vi "Main.vi"(9 "Tree Sync Refs":refnum<vi>[](array[refnum]), 10 "Tree Ref":refnum<vi>, 11 "Module Admin":refnum<class "Delacor_lib_QMH_Cloneable Module Admin.lvclass">) -> ()   [LabVIEW 2023, in "Tree Handlr.lvlib"]
doc: "This template is based off of the Queued Message Handler design pattern and the Queued Message Handler project template that ships with LabVIEW.\n\nThe main difference is that the queue is private to this module and communication between modules is performed via Broadcast and Request events.\n\nRequest events are wrapped in public API methods and are handled in the Event Handling Loop (EHL) of this VI. Any module can register for Broadcast events sent by this module. The EHL generates messages based on user interface actions.\n\nThe Message Handling Loop (MHL) processes messages generated by the EHL, or by other messages. The messages are string values, so new messages can be added easily to the Message Cases case structure in the MHL. Each message cluster can also provide an optional value for Message Data, which is a variant that can be converted to whatever message-specific data is required.\n_____\nBased on DQMH Project Template 7.0.1.1316."
uses:
  Tree Handlr.lvlib
  <vilib>/Delacor/Delacor QMH/Libraries/Cloneable Module Admin_class/Delacor_lib_QMH_Cloneable Module Admin.lvclass
  Module Data--cluster.ctl
  <vilib>/Delacor/Delacor QMH/Libraries/Message Queue_class/Delacor_lib_QMH_Message Queue.lvclass/Delacor_lib_QMH_Message Queue.ctl
  <vilib>/Delacor/Delacor QMH/Libraries/Cloneable Module Admin_class/Delacor_lib_QMH_Cloneable Module Admin.lvclass/Delacor_lib_QMH_Cloneable Module Admin.ctl
  Stop Argument--cluster.ctl
  <vilib>/Delacor/Delacor QMH/Libraries/Module Admin_class/Delacor_lib_QMH_Module Admin.lvclass/Delacor_lib_QMH_Module Admin.ctl
  Restore Open Items Argument--cluster.ctl
  <vilib>/Utility/miscctls.llb/LVPointTypeDef.ctl
  <vilib>/Delacor/Delacor QMH/Libraries/Message Queue_class/Delacor_lib_QMH_Enqueue Message (Multiline).vi
  <vilib>/Delacor/Delacor QMH/Libraries/Cloneable Module Admin_class/Delacor_lib_QMH_Get Module ID.vi
  <vilib>/Delacor/Delacor QMH/Libraries/Module Admin_class/Delacor_lib_QMH_Get External Launch.vi
  LabVIEW-common/TEMPLATES/State Machine/State Machine Sub/Process Multi-LineState String.vi
  <vilib>/Utility/inputDevices.llb/keyboardAcquire.vi
  <vilib>/Delacor/Delacor QMH/Libraries/Message Queue_class/Delacor_lib_QMH_Message Queue.lvclass
panel:
  out "error out":errorcluster
  out "Status":string
  in  "Simulate EHL Error":bool
  in  "Simulate MHL Error":bool
  # "Other processes communicate with this Module via its Public API (wrappers for its Request Events).\n\nThis Module communicates with other processes via its Broadcast Events.\nAny process that wants to receive these messages can register for this module's Broadcast events."
  # "This template is for the DQMH framework. See the block diagram for more information on how to use this template."
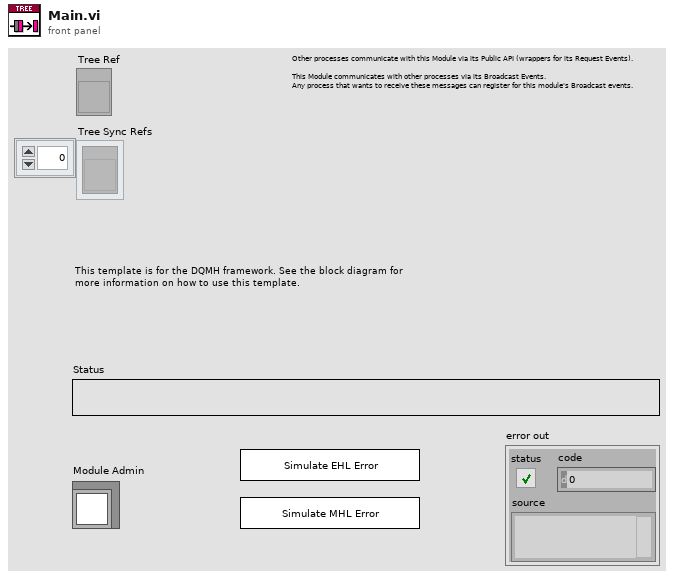
[diagram p1: front panel]
types:
  T1 = typedef "Tree Handlr.lvlib/Request Events--cluster.ctl" = cluster{"Stop Module":refnum<user-event>, "Show Panel":refnum<user-event>, "Hide Panel":refnum<user-event>, "Show Diagram":refnum<user-event>, "Get Module Execution Status":refnum<user-event>, "Restore Open Items":refnum<user-event>, "Record Open Items":refnum<user-event>}
  T2 = typedef "Tree Handlr.lvlib/Module Data--cluster.ctl" = cluster{"Status":string}
  T3 = enum32{"invalid lock state", "Not Locked", "Locked (No Password)", "Password-protected"}
  T4 = typedef "Tree Handlr.lvlib/Stop Argument--cluster.ctl" = cluster{"Module ID":i32, "Origin":string, "Exit via Stop Module Req?":bool, "Wait for Module to stop?":bool}
  T5 = enum16{"0", "1", "2", "3", "4", "5", "6", "7", "8", "9", "A", "B", "C", "D", "E", "F", "G", "H", "I", "J", "K", "L", "M", "N", "O", "P", "Q", "R", "S", "T", "U", "V", "W", "X", "Y", "Z", "F1", "F2", "F3", "F4", "F5", "F6", "F7", "F8", "F9", "F10", "F11", "F12", "F13", "F14", "F15", "ADD", "BACK", "BACKSLASH", "CAPITAL", "COMMA", "DECIMAL", "DELETE", "DIVIDE", "DOWN", "END", "EQUALS", "ESCAPE", "GRAVE (`)", "HOME", "INSERT", "LBRACKET", "LCONTROL", "LEFT", "L ALT", "LSHIFT", "LWIN", "MINUS", "MULTIPLY", "NEXT", "NUMLOCK", "NUMPAD_0", "NUMPAD_1", "NUMPAD_2", "NUMPAD_3", "NUMPAD_4", "NUMPAD_5", "NUMPAD_6", "NUMPAD_7", "NUMPAD_8", "NUMPAD_9", "PAUSE", "PERIOD", "PRIOR (PG UP)", "RBRACKET", "RCONTROL", "RETURN", "RIGHT", "R ALT", "RSHIFT", "RWIN", "SCROLL", "SEMICOLON", "SLASH", "SPACE", "SUBTRACT", "TAB", "UP", "ENTER (num pad)", "' (quote)"}
  T6 = typedef "Tree Handlr.lvlib/Restore Open Items Argument--cluster.ctl" = cluster{"Module ID":i32, "Boolean":bool}
  T7 = typedef "LVPointTypeDef.ctl" = cluster{"Horizontal":i16, "Vertical":i16}
  T8 = enum32{"Invalid", "Standard", "Closed", "Hidden", "Minimized", "Maximized"}
  T9 = enum16{"0", "1", "2", "3", "4", "5", "6", "7", "8", "9", "A", "B", "C", "D", "E", "F", "G", "H", "I", "J", "K", "L", "M", "N", "O", "P", "Q", "R", "S", "T", "U", "V", "W", "X", "Y", "Z", "F1", "F2", "F3", "F4", "F5", "F6", "F7", "F8", "F9", "F10", "F11", "F12", "F13", "F14", "F15", "ADD", "BACK", "BACKSLASH", "CAPITAL", "COMMA", "DECIMAL", "DELETE", "DIVIDE", "DOWN", "END", "EQUALS", "ESCAPE", "GRAVE (`)", "HOME", "INSERT", "LBRACKET", "LCONTROL", "LEFT", "L ALT", "LSHIFT", "LWIN", "MINUS", "MULTIPLY", "NEXT", "NUMLOCK", "NUMPAD_0", "NUMPAD_1", "NUMPAD_2", "NUMPAD_3", "NUMPAD_4", "NUMPAD_5", "NUMPAD_6", "NUMPAD_7", "NUMPAD_8", "NUMPAD_9", "PAUSE", "PERIOD", "PRIOR (PG UP)", "RBRACKET", "RCONTROL", "RETURN", "RIGHT", "R ALT", "RSHIFT", "RWIN", "SCROLL", "SEMICOLON", "SLASH", "SPACE", "SUBTRACT", "TAB", "UP", "ENTER (num pad)", "' (quote)"}[]
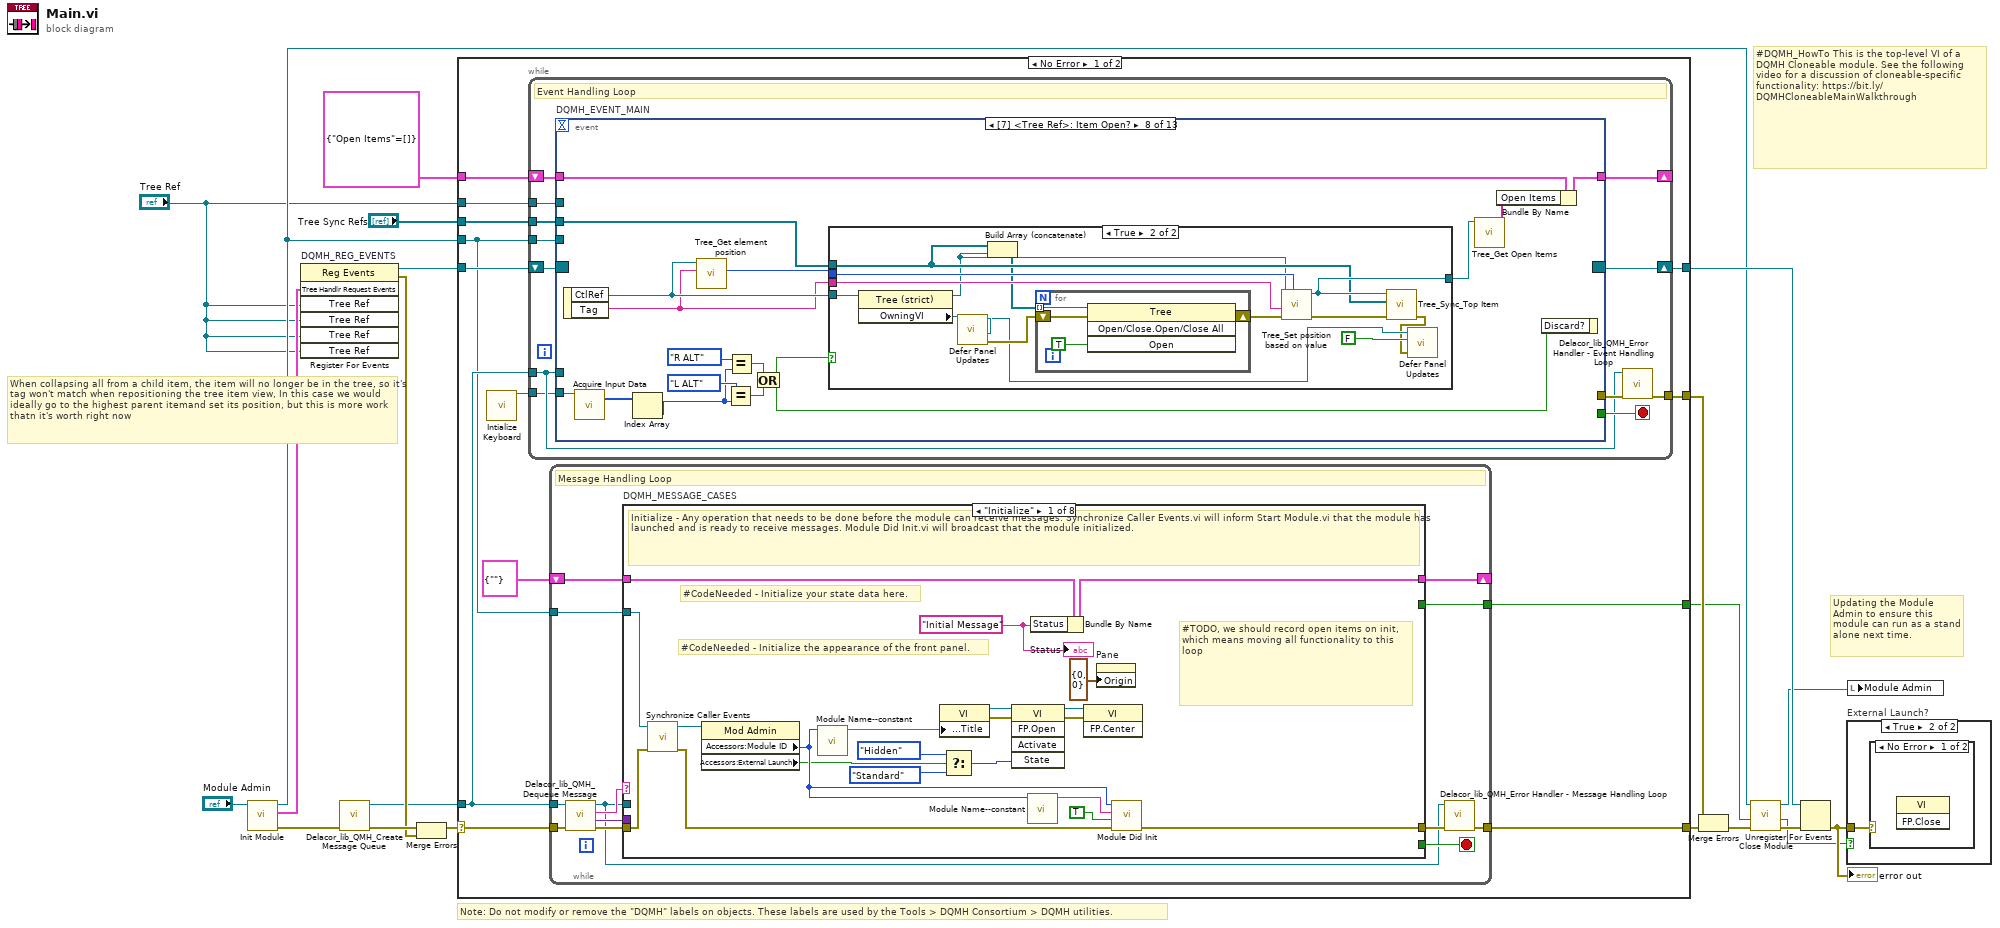
[diagram p0: block diagram]
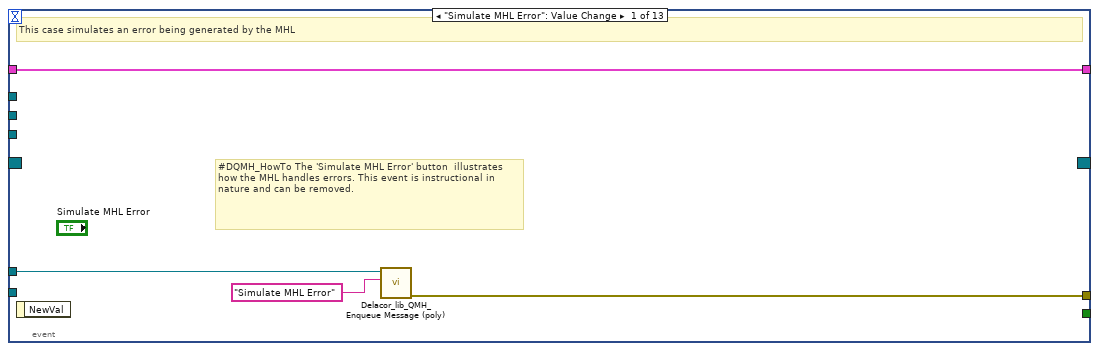
[diagram p2: hidden frame]
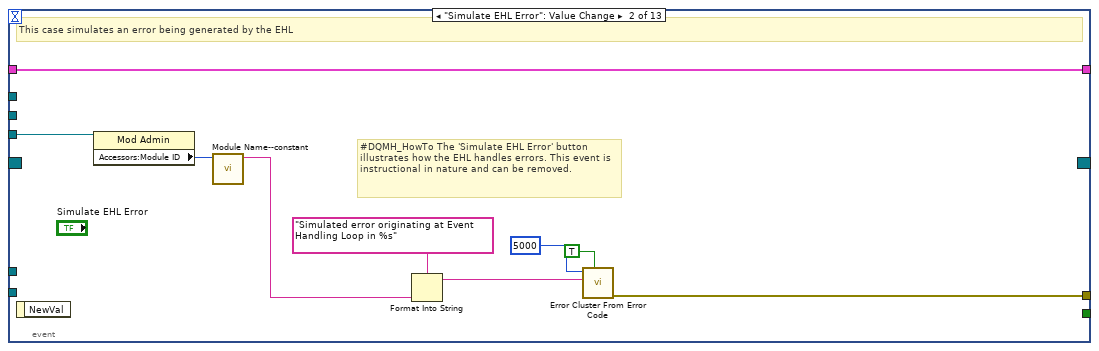
[diagram p3: hidden frame]
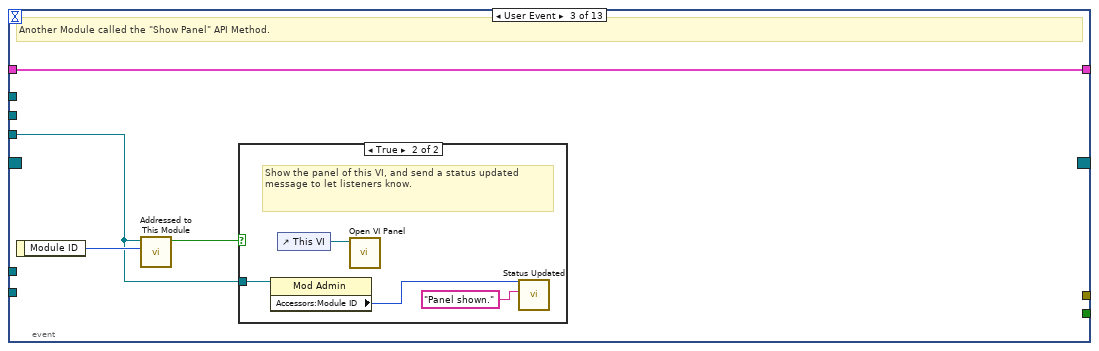
[diagram p4: hidden frame]
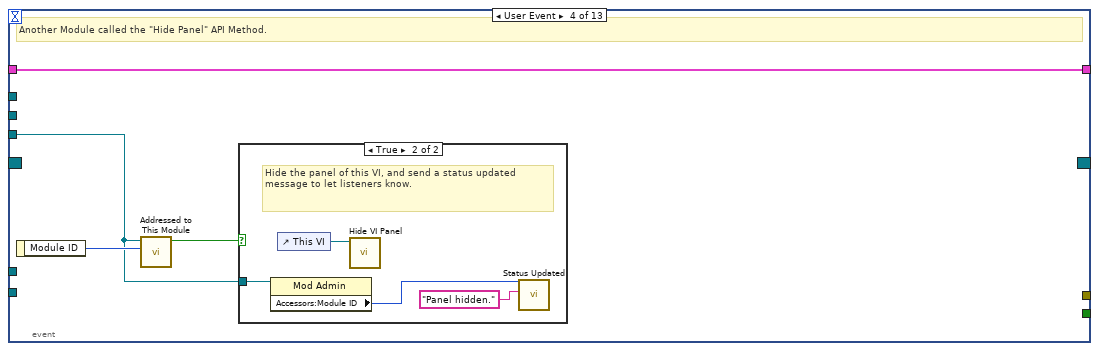
[diagram p6: hidden frame]
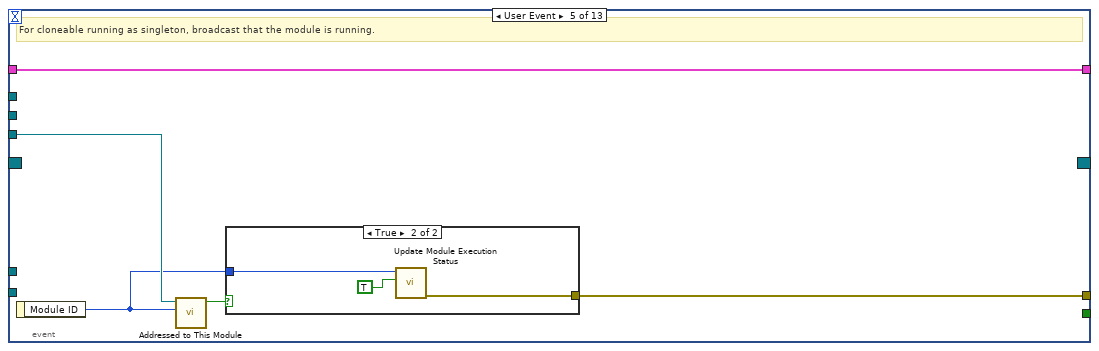
[diagram p8: hidden frame]
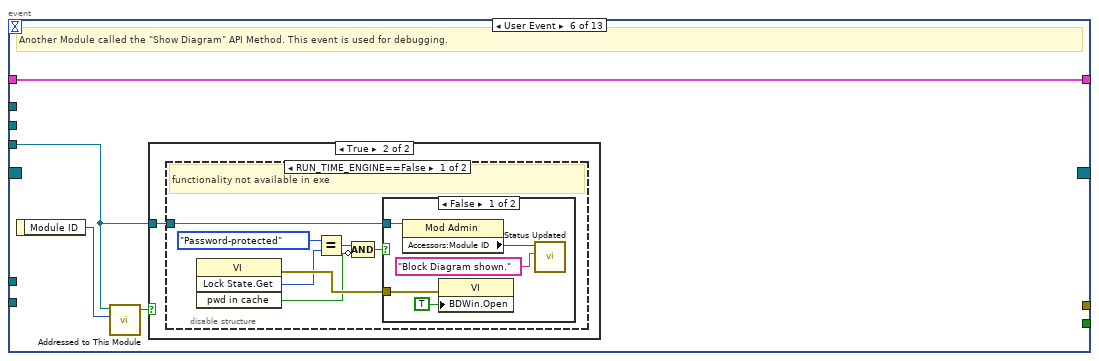
[diagram p10: hidden frame]
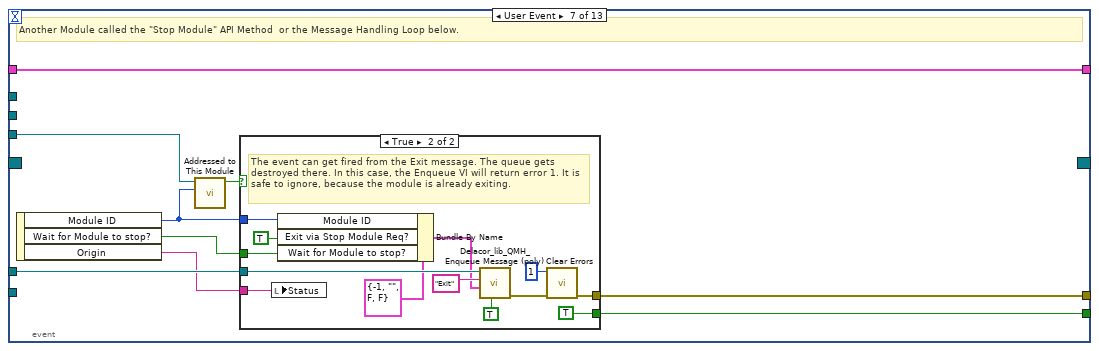
[diagram p14: hidden frame]
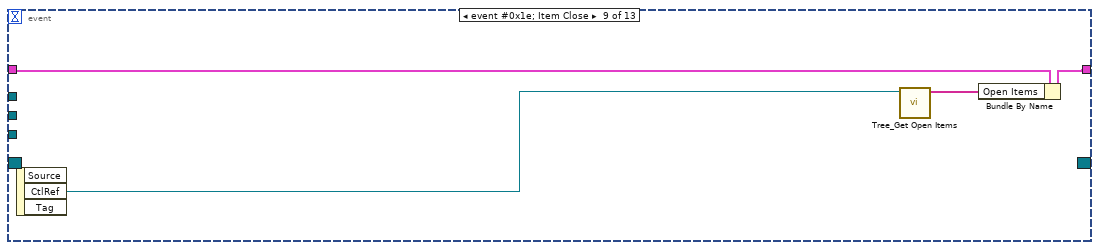
[diagram p17: hidden frame]
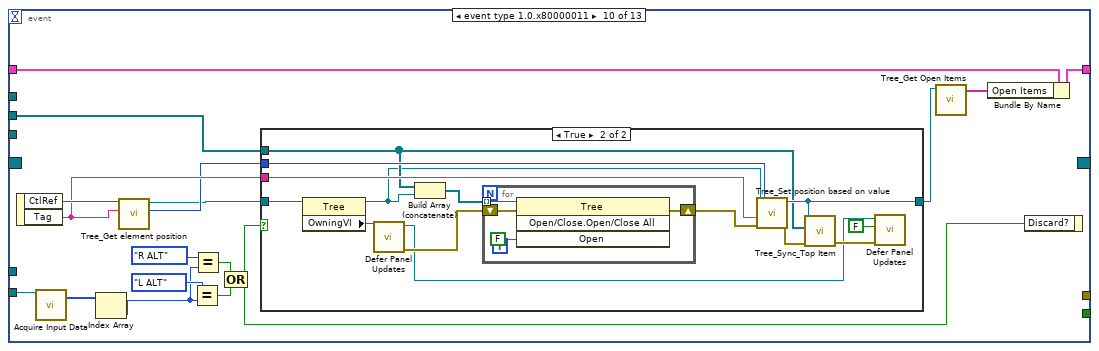
[diagram p18: hidden frame]
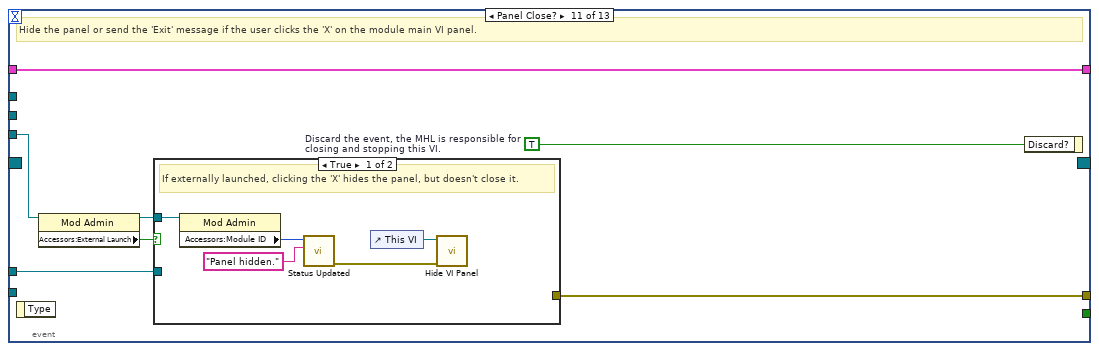
[diagram p20: hidden frame]
diagram:
  # "When collapsing all from a child item, the item will no longer be in the tree, so it's tag won't match when repositioning the tree item view, In this case we would ideally go to the highest parent itemand set its position, but this is more work thatn it's worth right now"
  # "#DQMH_HowTo This is the top-level VI of a DQMH Cloneable module. See the following video for a discussion of cloneable-specific functionality: https://bit.ly/DQMHCloneableMainWalkthrough"
  # "Note: Do not modify or remove the \"DQMH\" labels on objects. These labels are used by the Tools > DQMH Consortium > DQMH utilities."
  # "Updating the Module Admin to ensure this module can run as a stand alone next time."
  n1 = call "Init Module.vi"("Cloneable Module Admin in"="Module Admin") -> ("error out"=w18:errorcluster, "Tree Handlr Request Events"=w10:T1, "Cloneable Module Admin out"=w7:refnum<class "Delacor_lib_QMH_Cloneable Module Admin.lvclass">)  [unwired: 8 in]
  n2 = register-events "DQMH_REG_EVENTS"(w10, "Tree Ref", "Tree Ref", "Tree Ref", "Tree Ref") -> (reference out=w11:refnum<event-registration>, error out=w13:errorcluster)  [unwired: 2 in]
  n3 = call <vilib>:"Delacor_lib_QMH_Create Message Queue.vi"("error in"=w18) -> ("error out"=w15:errorcluster, "Message Queue"=w9:refnum<class "Delacor_lib_QMH_Message Queue.lvclass">)  [unwired: 9 in]
  n4 = Merge Errors(w15, w13) -> (w14:errorcluster)
  n5 = case shown="No Error" w14 {
    selector: w14 -> [w32 w347]
    tunnel: [w34 w346] -> w19
    tunnel: [w31 w345] -> w12
    tunnel: w11 -> [w29 w345]
    tunnel: w9 -> [w28 w338]
    tunnel: [w33 _] -> w20
    tunnel: w7 -> [w27 w341]
    tunnel: [w26 _] -> w5
    tunnel: cluster{"Open Items":string[]} {"Open Items"=[]} -> [w24 _]
    tunnel: "Tree Ref" -> [w23 _]
    tunnel: "Tree Sync Refs" -> [w22 _]
    frame No Error {
      n6 = call <vilib>:"Intialize Keyboard.vi"() -> ("device ID"=w25:refnum<k1>)  [unwired: 10 in, 1 out]
      n7 = while {
        tunnel: w28 -> [w40]
        shift-right: [w43] -> w31
        shift-left: w29 -> [w44]
        tunnel: [w45] -> w33
        tunnel: w27 -> [w41]
        tunnel: w25 -> [w39]
        shift-right: [w37] -> _
        shift-left: w24 -> [w38]
        tunnel: w23 -> [w36]
        tunnel: w22 -> [w35]
        stop <- w42 stop-if-true
        # "Event Handling Loop"
        n8 = event "DQMH_EVENT_MAIN" shown="[7] <Tree Ref>: Item Open?" {
          selector: w44 -> [_ _ _ _ _ _ _ _ _ _ _ _ _]
          dyn-events: [_ _ _ _ _ _ _ _ _ _ _ _ _] -> w43
          timeout: _ -> [_ _ _ _ _ _ _ _ _ _ _ _ _]
          tunnel: [_ _ _ _ _ _ w105 _ _ _ _ _ _] -> w42
          tunnel: w40 -> [w49 _ _ _ _ _ w108 _ _ _ w201 w223 _]
          tunnel: [w50 w59 _ _ w80 _ w109 _ _ _ w204 _ _] -> w46
          tunnel: w41 -> [_ w58 w61 w69 w78 w85 w107 _ _ _ w202 w221 w233]
          tunnel: w39 -> [_ _ _ _ _ _ _ w132 _ w172 _ _ _]
          tunnel: w38 -> [w47 w51 w60 w68 w76 w84 w101 w127 w161 w167 w198 w215 w231]
          tunnel: [w47 w51 w60 w68 w76 w84 w101 w126 w160 w166 w198 w214 w230] -> w37
          tunnel: w36 -> [_ _ _ _ _ _ _ _ _ _ _ w216 w229]
          tunnel: w35 -> [_ _ _ _ _ _ _ w123 _ w162 _ _ _]
          event "Simulate MHL Error": Value Change {
            # "#DQMH_HowTo The 'Simulate MHL Error' button  illustrates how the MHL handles errors. This event is instructional in nature and can be removed."
            # "This case simulates an error being generated by the MHL"
            n9 = event-data() -> ()  [unwired: 1 in, 1 out]
            n10 = call-poly <vilib>:"Delacor_lib_QMH_Enqueue Message (poly).vi"("Message"="Simulate MHL Error", "Message Queue in"=w49) -> ("error out"=w50:errorcluster)  [unwired: 8 in, 1 out]
          }
          event "Simulate EHL Error": Value Change {
            # "#DQMH_HowTo The 'Simulate EHL Error' button  illustrates how the EHL handles errors. This event is instructional in nature and can be removed."
            # "This case simulates an error being generated by the EHL"
            n11 = event-data() -> ()  [unwired: 1 in, 1 out]
            n12 = property on="Property Node" class="Mod Admin"(reference=w58) -> ("Accessors:Module ID"=w57:i32)  [unwired: 1 in, 2 out]
            n13 = call "Module Name--constant.vi"("Module ID"=w57) -> ("Module Name"=w52:string)  [unwired: 10 in]
            n14 = Format Into String(format string="Simulated error originating at Event Handling Loop in %s", w52) -> (resulting string=w55:string)  [unwired: 2 in, 1 out]
            n15 = call <vilib>:"Error Cluster From Error Code.vi"("show call chain? (False)"=TRUE, "error message (\"\")"=w55, "error code (0)"=5000) -> ("error out"=w59:errorcluster)  [unwired: 6 in]
          }
          event User Event {
            # "Another Module called the \"Show Panel\" API Method."
            n16 = event-data() -> ("Module ID"=w62:i32)  [unwired: 1 in]
            n17 = call "Addressed to This Module.vi"("Module ID from Argument"=w62, "Module Admin"=w61) -> ("Addressed to this instance?"=w63:bool)  [unwired: 8 in, 1 out]
            n18 = case shown="True" w63 {
              tunnel: w61 -> [_ w65]
              frame False {
              }
              frame True {
                # "Show the panel of this VI, and send a status updated message to let listeners know."
                n19 = property on="Property Node" class="Mod Admin"(reference=w65) -> ("Accessors:Module ID"=w64:i32)  [unwired: 1 in, 2 out]
                n20 = control-ref of="This VI"() -> (w67:refnum<vi>)
                n21 = call "Open VI Panel.vi"("VI"=w67) -> ()  [unwired: 10 in, 1 out]
                n22 = call "Status Updated.vi"("Status"="Panel shown." ("format string"), "Module ID"=w64) -> ()  [unwired: 9 in, 1 out]
              }
            }
          }
          event User Event {
            # "Another Module called the \"Hide Panel\" API Method."
            n23 = event-data() -> ("Module ID"=w70:i32)  [unwired: 1 in]
            n24 = call "Addressed to This Module.vi"("Module ID from Argument"=w70, "Module Admin"=w69) -> ("Addressed to this instance?"=w71:bool)  [unwired: 8 in, 1 out]
            n25 = case shown="True" w71 {
              tunnel: w69 -> [_ w73]
              frame False {
              }
              frame True {
                # "Hide the panel of this VI, and send a status updated message to let listeners know."
                n26 = property on="Property Node" class="Mod Admin"(reference=w73) -> ("Accessors:Module ID"=w72:i32)  [unwired: 1 in, 2 out]
                n27 = control-ref of="This VI"() -> (w75:refnum<vi>)
                n28 = call "Hide VI Panel.vi"("VI"=w75) -> ()  [unwired: 10 in, 1 out]
                n29 = call "Status Updated.vi"("Status"="Panel hidden." ("format string"), "Module ID"=w72) -> ()  [unwired: 9 in, 1 out]
              }
            }
          }
          event User Event {
            # "For cloneable running as singleton, broadcast that the module is running."
            n30 = event-data() -> ("Module ID"=w77:i32)  [unwired: 1 in]
            n31 = call "Addressed to This Module.vi"("Module ID from Argument"=w77, "Module Admin"=w78) -> ("Addressed to this instance?"=w79:bool)  [unwired: 8 in, 1 out]
            n32 = case shown="True" w79 {
              tunnel: [_ w83] -> w80
              tunnel: w77 -> [_ w82]
              frame False {
              }
              frame True {
                n33 = call "Update Module Execution Status.vi"("Running?"=TRUE, "Module ID"=w82) -> ("error out"=w83:errorcluster)  [unwired: 9 in]
              }
            }
          }
          event User Event {
            # "Another Module called the \"Show Diagram\" API Method. This event is used for debugging."
            n34 = event-data() -> ("Module ID"=w86:i32)  [unwired: 1 in]
            n35 = call "Addressed to This Module.vi"("Module ID from Argument"=w86, "Module Admin"=w85) -> ("Addressed to this instance?"=w87:bool)  [unwired: 8 in, 1 out]
            n36 = case shown="True" w87 {
              tunnel: w85 -> [_ w88]
              frame False {
              }
              frame True {
                n37 = disable-structure shown="RUN_TIME_ENGINE==False" {
                  disable-tunnel: w88 -> [w89 _]
                  frame condition #0 (active) {
                    # "functionality not available in exe"
                    n38 = invoke on="Invoke Node" class="VI" method="Lock State.Get"() -> (error out=w95:errorcluster, "Get Lock State"=w94:T3, "pwd in cache"=w91:bool)  [unwired: 4 in, 1 out]
                    n39 = Equal?(x=T3."Password-protected", y=w94) -> (x = y?=w92:bool)
                    n40 = Compound Arithmetic op=AND(w92, invert w91) -> (w90:bool)
                    n41 = case shown="False" w90 {
                      tunnel: w95 -> [w100 _]
                      tunnel: w89 -> [w97 _]
                      frame False {
                        n42 = property on="Property Node" class="Mod Admin"(reference=w97) -> ("Accessors:Module ID"=w96:i32)  [unwired: 1 in, 2 out]
                        n43 = property on="Property Node" class="VI"(error in=w100, "BDWin.Open"=TRUE ("Block Diagram Window:Open")) -> ()  [unwired: 1 in, 2 out]
                        n44 = call "Status Updated.vi"("Status"="Block Diagram shown." ("format string"), "Module ID"=w96) -> ()  [unwired: 9 in, 1 out]
                      }
                      frame True {
                        # "Password-protected VI, and the password is not in the cache. Do not show the diagram."
                      }
                    }
                  }
                  frame condition #1 {
                  }
                }
              }
            }
          }
          event User Event {
            # "Another Module called the \"Stop Module\" API Method  or the Message Handling Loop below."
            n45 = event-data() -> ("Module ID"=w103:i32, "Wait for Module to stop?"=w104:bool, "Origin"=w102:string)  [unwired: 1 in]
            n46 = call "Addressed to This Module.vi"("Module ID from Argument"=w103, "Module Admin"=w107) -> ("Addressed to this instance?"=w106:bool)  [unwired: 8 in, 1 out]
            n47 = case shown="True" w106 {
              tunnel: [_ w121] -> w109
              tunnel: w108 -> [_ w117]
              tunnel: [_ TRUE] -> w105
              tunnel: w104 -> [_ w112]
              tunnel: w103 -> [_ w114]
              tunnel: w102 -> [_ w110]
              frame False {
              }
              frame True {
                # "The event can get fired from the Exit message. The queue gets destroyed there. In this case, the Enqueue VI will return error 1. It is safe to ignore, because the module is already exiting."
                n48 = local write "Status"(w110) -> ()
                n49 = Bundle By Name(cluster=T4 {"Module ID"=-1, "Origin"="", "Exit via Stop Module Req?"=FALSE, "Wait for Module to stop?"=FALSE} ("Stop Argument"), "Module ID"=w114, "Exit via Stop Module Req?"=TRUE, "Wait for Module to stop?"=w112) -> (w111:T4)
                n50 = call-poly <vilib>:"Delacor_lib_QMH_Enqueue Message (poly).vi"("Priority Message? (F)"=TRUE, "Message Data"=w111, "Message"="Exit", "Message Queue in"=w117) -> ("error out"=w122:errorcluster)  [unwired: 6 in, 1 out]
                n51 = call <vilib>:"Clear Errors.vi"("error in (no error)"=w122, "specific error code to clear (0: all)"=1) -> ("error out"=w121:errorcluster)  [unwired: 4 in, 1 out]
              }
            }
          }
          event Item Open? {
            n52 = event-data() -> ("CtlRef"=w130:refnum<vi>, "Tag"=w129:string)  [unwired: 1 in]
            n53 = call-poly <vilib>:"Acquire Input Data.vi"("device ID"=w132) -> ("keys pressed"=w138:T9)  [unwired: 16 in, 2 out]
            n54 = Index Array(array=w138) -> (element=w135:T5)  [unwired: 1 in]
            n55 = call "Tree_Get element position.vi"("tag"=w129, "Tree Ref In"=w130) -> ("Tree Item Row"=w128:i32)  [unwired: 7 in, 2 out]
            n56 = Equal?(x=T5."L ALT" ("element"), y=w135) -> (x = y?=w133:bool)
            n57 = Equal?(x=T5."R ALT" ("element"), y=w135) -> (x = y?=w134:bool)
            n58 = Compound Arithmetic op=OR(w134, w133) -> (w131:bool)
            n59 = case shown="True" w131 {
              tunnel: w129 -> [_ w153]
              tunnel: w130 -> [w139 w149]
              tunnel: w128 -> [_ w146]
              tunnel: [w139 w143] -> w124
              tunnel: w123 -> [_ w142]
              frame False {
              }
              frame True {
                n60 = property class="Tree (strict)"(reference=w149) -> (reference out=w140:refnum<vi>, "OwningVI"=w148:refnum<vi>)  [unwired: 1 in, 1 out]
                n61 = call "Defer Panel Updates.vi"("VI Ref"=w148) -> ("error out"=w151:errorcluster, "VI Ref Out"=w147:refnum<vi>)  [unwired: 9 in]
                n62 = Build Array (concatenate)(w142, w140) -> (w141:refnum<vi>[])
                n63 = for {
                  shift-right: [w155] -> w150
                  shift-left: w151 -> [w156]
                  tunnel: w141 -> [w154] mode=indexing
                  n64 = invoke class="Tree" method="Open/Close.Open/Close All"(reference=w154, error in=w156, "Open"=TRUE ("Open?")) -> (error out=w155:errorcluster)  [unwired: 1 in, 3 out]
                }
                n65 = call "Tree_Set position based on value.vi"("Set Position [-1, in range]"=w146, "error in (no error)"=w150, "tag"=w153, "Tree Ref"=w140) -> ("error out"=w145:errorcluster, "Tree Ref"=w143:refnum<vi>)  [unwired: 6 in]
                n66 = call "Tree_Sync_Top Item.vi"("error in"=w145, "All Tree Control Refs"=w142, "Changed Tree Control Ref"=w143) -> ("error out"=w144:errorcluster)  [unwired: 8 in]
                n67 = call "Defer Panel Updates.vi"("error in (no error)"=w144, "Defer Panel Updates [T]"=FALSE, "VI Ref"=w147) -> ()  [unwired: 7 in, 2 out]
              }
            }
            n68 = call "Tree_Get Open Items.vi"("Tree Ref"=w124) -> ("Open Tree Item Tags"=w125:string[])  [unwired: 10 in]
            n69 = Bundle By Name(cluster=w127, "Open Items"=w125) -> (w126:cluster{"Open Items":string[]})
            n70 = event-data("Discard?"=w131) -> ()  [unwired: 1 in, 1 out]
          }
          event event #0x1e; Item Close {
            n71 = event-data() -> ("CtlRef"=w158:refnum<vi>)  [unwired: 1 in, 2 out]
            n72 = call "Tree_Get Open Items.vi"("Tree Ref"=w158) -> ("Open Tree Item Tags"=w159:string[])  [unwired: 10 in]
            n73 = Bundle By Name(cluster=w161, "Open Items"=w159) -> (w160:cluster{"Open Items":string[]})
          }
          event event type 1.0.x80000011 {
            n74 = event-data() -> ("CtlRef"=w170:refnum<vi>, "Tag"=w169:string)  [unwired: 1 in]
            n75 = call-poly <vilib>:"Acquire Input Data.vi"("device ID"=w172) -> ("keys pressed"=w178:T9)  [unwired: 16 in, 2 out]
            n76 = Index Array(array=w178) -> (element=w175:T5)  [unwired: 1 in]
            n77 = call "Tree_Get element position.vi"("tag"=w169, "Tree Ref In"=w170) -> ("Tree Item Row"=w168:i32, "Tree Ref Out"=w164:refnum<vi>)  [unwired: 7 in, 1 out]
            n78 = Equal?(x=T5."L ALT" ("element"), y=w175) -> (x = y?=w173:bool)
            n79 = Equal?(x=T5."R ALT" ("element"), y=w175) -> (x = y?=w174:bool)
            n80 = Compound Arithmetic op=OR(w174, w173) -> (w171:bool)
            n81 = case shown="True" w171 {
              tunnel: w169 -> [_ w191]
              tunnel: w168 -> [_ w190]
              tunnel: w164 -> [w179 w189]
              tunnel: [w179 w184] -> w163
              tunnel: w162 -> [_ w182]
              frame False {
              }
              frame True {
                n82 = property class="Tree"(reference=w189) -> (reference out=w180:refnum<vi>, "OwningVI"=w188:refnum<vi>)  [unwired: 1 in, 1 out]
                n83 = call "Defer Panel Updates.vi"("VI Ref"=w188) -> ("error out"=w193:errorcluster, "VI Ref Out"=w183:refnum<vi>)  [unwired: 9 in]
                n84 = Build Array (concatenate)(w182, w180) -> (w181:refnum<vi>[])
                n85 = for {
                  shift-right: [w195] -> w187
                  shift-left: w193 -> [w196]
                  tunnel: w181 -> [w194] mode=indexing
                  n86 = invoke class="Tree" method="Open/Close.Open/Close All"(reference=w194, error in=w196, "Open"=FALSE ("Open?")) -> (error out=w195:errorcluster)  [unwired: 1 in, 3 out]
                }
                n87 = call "Tree_Set position based on value.vi"("Set Position [-1, in range]"=w190, "error in (no error)"=w187, "tag"=w191, "Tree Ref"=w180) -> ("error out"=w186:errorcluster, "Tree Ref"=w184:refnum<vi>)  [unwired: 6 in]
                n88 = call "Tree_Sync_Top Item.vi"("error in"=w186, "All Tree Control Refs"=w182, "Changed Tree Control Ref"=w184) -> ("error out"=w185:errorcluster)  [unwired: 8 in]
                n89 = call "Defer Panel Updates.vi"("error in (no error)"=w185, "Defer Panel Updates [T]"=FALSE, "VI Ref"=w183) -> ()  [unwired: 7 in, 2 out]
              }
            }
            n90 = call "Tree_Get Open Items.vi"("Tree Ref"=w163) -> ("Open Tree Item Tags"=w165:string[])  [unwired: 10 in]
            n91 = Bundle By Name(cluster=w167, "Open Items"=w165) -> (w166:cluster{"Open Items":string[]})
            n92 = event-data("Discard?"=w171) -> ()  [unwired: 1 in, 1 out]
          }
          event Panel Close? {
            w203 = TRUE  # Discard the event, the MHL is responsible for closing and stopping this VI.
            # "Hide the panel or send the 'Exit' message if the user clicks the 'X' on the module main VI panel."
            n93 = event-data() -> ()  [unwired: 1 in, 1 out]
            n94 = property on="Property Node" class="Mod Admin"(reference=w202) -> (reference out=w199:refnum<class "Delacor_lib_QMH_Cloneable Module Admin.lvclass">, "Accessors:External Launch"=w200:bool)  [unwired: 1 in, 1 out]
            n95 = case shown="True" w200 {
              tunnel: w201 -> [_ w212]
              tunnel: [_ w213] -> w204
              tunnel: w199 -> [w207 _]
              frame True {
                # "If externally launched, clicking the 'X' hides the panel, but doesn't close it."
                n96 = property on="Property Node" class="Mod Admin"(reference=w207) -> ("Accessors:Module ID"=w206:i32)  [unwired: 1 in, 2 out]
                n97 = call "Status Updated.vi"("Status"="Panel hidden." ("format string"), "Module ID"=w206) -> ("error out"=w205:errorcluster)  [unwired: 9 in]
                n98 = control-ref of="This VI"() -> (w209:refnum<vi>)
                n99 = call "Hide VI Panel.vi"("error in"=w205, "VI"=w209) -> ()  [unwired: 9 in, 1 out]
              }
              frame False {
                # "If run as a stand-alone VI, clicking the panel 'X' stops the VI."
                n100 = call-poly <vilib>:"Delacor_lib_QMH_Enqueue Message (poly).vi"("Priority Message? (F)"=TRUE, "Message"="Exit", "Message Queue in"=w212) -> ("error out"=w213:errorcluster)  [unwired: 7 in, 1 out]
              }
            }
            n101 = event-data ("Event Filter Node")("Discard?"=w203) -> ()  [unwired: 1 in, 1 out]
          }
          event User Event {
            # "Another Module called the \"Restore Open Items\" API Method."
            n102 = event-data() -> ("Module ID"=w218:i32, "Boolean"=w217:bool)  [unwired: 1 in]
            n103 = Bundle(cluster=T6 {"Module ID"=-1, "Boolean"=FALSE} ("Restore Open Items Argument"), "Module ID"=w218, "Boolean"=w217) -> (w219:T6)
            n104 = call "Addressed to This Module.vi"("Module ID from Argument"=w218, "Module Admin"=w221) -> ("Addressed to this instance?"=w222:bool)  [unwired: 8 in, 1 out]
            n105 = case shown="True" w222 {
              tunnel: w223 -> [_ _]
              tunnel: w219 -> [_ _]
              tunnel: w216 -> [_ w227]
              tunnel: w215 -> [w224 w225]
              tunnel: [w224 w225] -> w214
              frame False {
              }
              frame True {
                n106 = Unbundle By Name(w225) -> ("Open Items"=w226:string[])
                n107 = call "Tree_Set Open Items.vi"("Open Tree Item Tags"=w226, "Tree Ref"=w227) -> ()  [unwired: 10 in]
              }
            }
          }
          event User Event {
            # "Another Module called the \"Record Open Items\" API Method."
            n108 = event-data() -> ("Module ID"=w232:i32)  [unwired: 1 in, 1 out]
            n109 = call "Addressed to This Module.vi"("Module ID from Argument"=w232, "Module Admin"=w233) -> ("Addressed to this instance?"=w228:bool)  [unwired: 8 in, 1 out]
            n110 = case shown="True" w228 {
              tunnel: w231 -> [w234 w237]
              tunnel: [w234 w236] -> w230
              tunnel: w229 -> [_ w235]
              frame False {
              }
              frame True {
                n111 = call "Tree_Get Open Items.vi"("Tree Ref"=w235) -> ("Open Tree Item Tags"=w238:string[])  [unwired: 10 in]
                n112 = Bundle By Name(cluster=w237, "Open Items"=w238) -> (w236:cluster{"Open Items":string[]})
              }
            }
          }
        }
        n113 = call-dynamic "Delacor_lib_QMH_Error Handler - Event Handling Loop.vi"("error in"=w46, "Message Queue in"=w40) -> ("dup error in"=w45:errorcluster)  [unwired: 8 in, 1 out]
      }
      n114 = while {
        tunnel: w28 -> [w239]
        shift-right: [w246] -> _
        shift-left: T2 {"Status"=""} ("Data Cluster") -> [w247]
        tunnel: w32 -> [w250]
        tunnel: [w248] -> w34
        tunnel: w27 -> [w241]
        tunnel: [w240] -> w26
        stop <- w245 stop-if-true
        # "Message Handling Loop"
        n115 = call-dynamic "Delacor_lib_QMH_Dequeue Message.vi"("error in"=w250, "Message Queue in"=w239) -> ("error out"=w249:errorcluster, "Message Data"=w243:variant, "Message"=w244:string, "Message Queue out"=w242:refnum<class "Delacor_lib_QMH_Message Queue.lvclass">)  [unwired: 6 in]
        n116 = case "DQMH_MESSAGE_CASES" shown="\"Initialize\"" w244 {
          selector: w244 -> [_ _ _ _ _ _ _ w327]
          tunnel: w242 -> [_ _ _ _ w282 _ w319 _]
          tunnel: w249 -> [w270 w274 w277 w279 w291 w308 w325 w336]
          tunnel: [w268 w274 w276 w279 w287 w307 w320 w337] -> w251
          tunnel: w247 -> [w261 w273 w275 w278 w286 w305 w318 w334]
          tunnel: [w260 w273 w275 w278 w286 w305 w318 w334] -> w246
          tunnel: [_ _ _ _ _ _ w317 _] -> w245
          tunnel: w243 -> [_ _ _ _ w285 _ w315 _]
          tunnel: w241 -> [w255 _ _ _ w284 w303 w310 w333]
          tunnel: [_ _ _ _ _ _ w313 _] -> w240
          frame "Initialize" {
            w252 = "Initial Message" ("Initial Message")
            # "#TODO, we should record open items on init, which means moving all functionality to this loop"
            # "#CodeNeeded - Initialize the appearance of the front panel."
            # "#CodeNeeded - Initialize your state data here."
            # "Initialize - Any operation that needs to be done before the module can receive messages. Synchronize Caller Events.vi will inform Start Module.vi that the module has launched and is ready to receive messages. Module Did Init.vi will broadcast that the module initialized."
            n117 = call "Synchronize Caller Events.vi"("error in"=w270, "Module Admin"=w255) -> ("error out"=w269:errorcluster, "Module Admin out"=w254:refnum<class "Delacor_lib_QMH_Cloneable Module Admin.lvclass">)  [unwired: 8 in]
            n118 = property on="Property Node" class="Mod Admin"(reference=w254) -> ("Accessors:Module ID"=w257:i32, "Accessors:External Launch"=w256:bool)  [unwired: 1 in, 2 out]
            n119 = call "Module Name--constant.vi"("Module ID"=w257) -> ("Module Name"=w265:string)  [unwired: 10 in]
            n120 = property on="Property Node" class="VI"("Front Panel.Title"=w265) -> (reference out=w267:refnum<vi>, error out=w272:errorcluster)  [unwired: 2 in]
            n121 = Select(t=T8."Hidden" ("State"), s=w256, f=T8."Standard" ("State")) -> (s? t:f=w262:T8)
            n122 = invoke on="Invoke Node" class="VI" method="FP.Open"(reference=w267, error in=w272, "State"=w262) -> (reference out=w266:refnum<vi>, error out=w271:errorcluster)  [unwired: 2 in, 3 out]
            n123 = call "Module Name--constant.vi"("Module ID"=w257) -> ("Module Name"=w258:string)  [unwired: 10 in]
            n124 = Bundle By Name(cluster=w261, "Status"=w252) -> (w260:T2)
            n125 = invoke on="Invoke Node" class="VI" method="FP.Center"(reference=w266, error in=w271) -> ()  [unwired: 1 in, 3 out]
            n126 = property on="Pane" class="Pane"("Origin"=T7 {"Horizontal"=0, "Vertical"=0}) -> ()  [unwired: 2 in, 2 out]
            n127 = call "Module Did Init.vi"("error in"=w269, "Initialized?"=TRUE, "Origin"=w258, "Module ID"=w257) -> ("error out"=w268:errorcluster)  [unwired: 7 in]
            "Status" <- w252
          }
          frame "---Module Specific---" {
            # "Separator -- The following cases handle messages specific to this Module."
          }
          frame "---Copy This Frame---" {
            # "Duplicate this frame when creating new messages.  Change this comment in the duplicated frame to describe this message."
            n128 = Merge Errors(w277) -> (w276:errorcluster)
          }
          frame "---Exit and Error Handling---" {
            # "Separator - the following cases handle errors and exit messages."
          }
          frame "Error" {
            # "#CodeRecommended - If the module is running in standalone mode (External Launch = FALSE), this code will pop up an error dialog and call the 'Exit' message if an error occurs. Add more fine-grained error management here."
            # "Error - Check the error message data and respond accordingly. This message is sent by the \"Error Handler\" VIs at the end of each loop in this application."
            n129 = property on="Property Node" class="Mod Admin"(reference=w284) -> ("Accessors:External Launch"=w283:bool, "Accessors:Module ID"=w281:i32)  [unwired: 1 in, 2 out]
            n130 = Variant To Data(error in=w291, type=errorcluster {"status"=FALSE, "code"=0, "source"=""} ("error constant"), Variant=w285) -> (data=w280:errorcluster, error out=w289:errorcluster)
            n131 = local write "error out"(w280) -> ()
            n132 = call "Error Reported.vi"("Error"=w280, "Module ID"=w281) -> ()  [unwired: 9 in, 1 out]
            n133 = case shown="True" w283 {
              tunnel: [w296 _] -> w288
              tunnel: w282 -> [w294 _]
              tunnel: w280 -> [w295 _]
              frame False {
                n134 = disable-structure shown="Default" {
                  disable-tunnel: w295 -> [w297 _]
                  frame condition #0 (active) {
                    # "If the module is running standalone, then pop up an error dialog and call the \"Exit\" message."
                    n135 = call <vilib>:"Simple Error Handler.vi"("error in (no error)"=w297) -> ()  [unwired: 4 in, 5 out]
                  }
                  frame condition #1 {
                    # "To prevent the Simple Error Handler VI from being loaded (e.g. when deploying to a Real-Time target), add the Conditional Disable Symbol \"DQMH_Disable_SEH\" to your project and set it to TRUE."
                  }
                }
                n136 = call-poly <vilib>:"Delacor_lib_QMH_Enqueue Message (poly).vi"("Priority Message? (F)"=TRUE, "Message"="Exit", "Message Queue in"=w294) -> ("error out"=w296:errorcluster)  [unwired: 7 in, 1 out]
              }
              frame True {
                # "If the module was launched externally, calling the Error Reported broadcast VI is the only action performed by the \"Error\" message. The module's caller can then process the error appropriately."
              }
            }
            n137 = Merge Errors(w289, w288) -> (w287:errorcluster)
          }
          frame "Simulate MHL Error" {
            # "#DQMH_HowTo The 'Simulate MHL Error' button  illustrates how the MHL handles errors. This event is instructional in nature and can be removed."
            # "Simulate an error occurring at the MHL"
            n138 = property on="Property Node" class="Mod Admin"(reference=w303) -> ("Accessors:Module ID"=w304:i32)  [unwired: 1 in, 2 out]
            n139 = call "Module Name--constant.vi"("Module ID"=w304) -> ("Module Name"=w299:string)  [unwired: 10 in]
            n140 = Format Into String(format string="Simulated error originating at Message Handling Loop in %s", w299) -> (resulting string=w300:string)  [unwired: 2 in, 1 out]
            n141 = call <vilib>:"Error Cluster From Error Code.vi"("show call chain? (False)"=TRUE, "error message (\"\")"=w300, "error code (0)"=5001) -> ("error out"=w306:errorcluster)  [unwired: 6 in]
            n142 = Merge Errors(w308, w306) -> (w307:errorcluster)
          }
          frame "Exit" {
            w316 = 91  # 91: not all Exit messages will have an argument
            w317 = TRUE  # Stop the VI
            # "Release the message queue reference"
            # "#CodeNeeded - Add any required cleanup code here."
            # "Exit - Exit the application."
            n143 = Variant To Data(error in=w325, type=T4 {"Module ID"=-1, "Origin"="", "Exit via Stop Module Req?"=FALSE, "Wait for Module to stop?"=FALSE} ("Stop Argument"), Variant=w315) -> (data=w312:T4, error out=w321:errorcluster)
            n144 = call <vilib>:"Clear Errors.vi"("error in (no error)"=w321, "specific error code to clear (0: all)"=w316) -> ("error out"=w324:errorcluster)  [unwired: 4 in, 1 out]
            n145 = property on="Property Node" class="Mod Admin"(reference=w310) -> ("Accessors:Module ID"=w309:i32)  [unwired: 1 in, 2 out]
            n146 = control-ref of="This VI"() -> (w311:refnum<vi>)
            n147 = call-dynamic "Delacor_lib_QMH_Release Message Queue.vi"("error in"=w324, "Message Queue"=w319) -> ("error out"=w323:errorcluster)  [unwired: 9 in]
            n148 = call "Handle Exit.vi"("Stop Argument"=w312, "Module Admin in"=w310, "VI reference"=w311) -> ("error out"=w322:errorcluster, "Wait for Stop?"=w313:bool)  [unwired: 7 in]
            n149 = Merge Errors(w323, w322) -> (w320:errorcluster)
            n150 = call "Error Reported.vi"("Error"=w320, "Module ID"=w309) -> ()  [unwired: 9 in, 1 out]
          }
          frame Default {
            # "'Default' case only runs if there is a message that isn't defined in any of the other cases.  Output a programming error."
            n151 = property on="Property Node" class="Mod Admin"(reference=w333) -> ("Accessors:Module ID"=w332:i32)  [unwired: 1 in, 2 out]
            n152 = call "Module Name--constant.vi"("Module ID"=w332) -> ("Module Name"=w326:string)  [unwired: 10 in]
            n153 = Format Into String(format string="The invalid message string \"%s\" was received in the Message Handling Loop for module \"%s\".", w327, w326) -> (resulting string=w329:string)  [unwired: 2 in, 1 out]
            n154 = call <vilib>:"Error Cluster From Error Code.vi"("show call chain? (False)"=TRUE, "error message (\"\")"=w329, "error code (0)"=1) -> ("error out"=w335:errorcluster)  [unwired: 6 in]
            n155 = Merge Errors(w336, w335) -> (w337:errorcluster)
          }
        }
        n156 = call-dynamic "Delacor_lib_QMH_Error Handler - Message Handling Loop.vi"("error in"=w251, "Message Queue in"=w242) -> ("dup error in"=w248:errorcluster)  [unwired: 8 in, 1 out]
      }
    }
    frame Error {
      n157 = call "Synchronize Caller Events.vi"("Module Admin"=w341) -> ("Module Admin out"=w340:refnum<class "Delacor_lib_QMH_Cloneable Module Admin.lvclass">)  [unwired: 9 in, 1 out]
      n158 = property on="Property Node" class="Mod Admin"(reference=w340) -> ("Accessors:Module ID"=w339:i32)  [unwired: 1 in, 2 out]
      n159 = call-dynamic "Delacor_lib_QMH_Release Message Queue.vi"("error in"=w347, "Message Queue"=w338) -> ("error out"=w346:errorcluster)  [unwired: 9 in]
      n160 = call "Module Name--constant.vi"("Module ID"=w339) -> ("Module Name"=w344:string)  [unwired: 10 in]
      n161 = Format Into String(format string="An error occurred during initialization. %s is no longer running.", w344) -> (resulting string=w342:string)  [unwired: 2 in, 1 out]
      n162 = call "Error Reported.vi"("Additional Information"=w342, "Error"=w346, "Module ID"=w339) -> ()  [unwired: 8 in, 1 out]
    }
  }
  n163 = Merge Errors(w20, w19) -> (w21:errorcluster)
  n164 = call "Close Module.vi"("error in"=w21, "Wait for stop?"=w5, "Module Admin in"=w7) -> ("error out"=w17:errorcluster, "External Launch"=w4:bool, "Module Admin out"=w6:refnum<class "Delacor_lib_QMH_Cloneable Module Admin.lvclass">)  [unwired: 6 in]
  n165 = Unregister For Events(event registration refnum=w12, error in=w17) -> (error out=w16:errorcluster)
  "error out" <- w16
  n166 = case "External Launch?" shown="True" w4 {
    tunnel: w16 -> [_ w348]
    frame False {
    }
    frame True {
      n167 = case shown="No Error" w348 {
        frame No Error {
          n168 = invoke class="VI" method="FP.Close"() -> ()  [unwired: 3 in, 3 out]
        }
        frame Error {
          n169 = invoke class="VI" method="FP.Open"("Activate"=TRUE ("Activate?")) -> ()  [unwired: 4 in, 5 out]
        }
      }
    }
  }
  n170 = local write "Module Admin"(w6) -> ()
